vi "onCreateListener.vi"(6 "timeout (ms)":i32=100, 8 "error in (no error)":errorcluster, 10 "Configuration":refnum<class "Connection.TCP-TLS.lvclass">) -> (0 "error out":errorcluster, 3 "Listener":refnum<class "Connection.lvclass">)   [LabVIEW 2020, in "Connection.TCP-TLS.lvclass"]
uses:
  Connection.TCP-TLS.lvclass
  Connection.TCP-TLS.lvclass/Connection.TCP-TLS.ctl
  <vilib>/LabVIEW Open Source Project/MQTT TCP Connection/MQTT_TCP/Connection/TCPConnection.lvclass
  C:/Program Files (x86)/National Instruments/LabVIEW 2020/vi.lib/LabVIEW Open Source Project/MQTT TCP Connection/MQTT_TCP/Connection/TCPConnection.lvclass
  C:/Program Files (x86)/National Instruments/LabVIEW 2020/vi.lib/LabVIEW Open Source Project/MQTT Connection/MQTT_Connection/Connection/Connection.lvclass
  C:/Program Files (x86)/National Instruments/LabVIEW 2020/vi.lib/LabVIEW Open Source Project/Connection/Connection/Connection.lvclass
  C:/Repositories/LVOS/MQTT-Connection-SecuredTCP/source/Connection.SecuredTCP/Connection.TCP-TLS.lvclass
  <vilib>/LabVIEW Open Source Project/Connection/Connection/Connection.lvclass
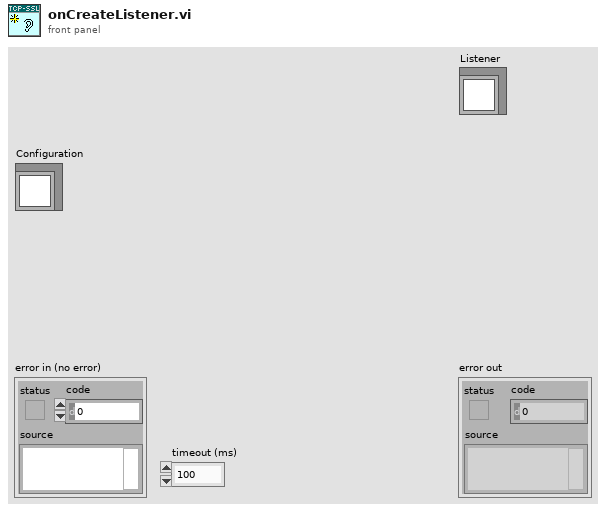
[diagram p1: front panel]
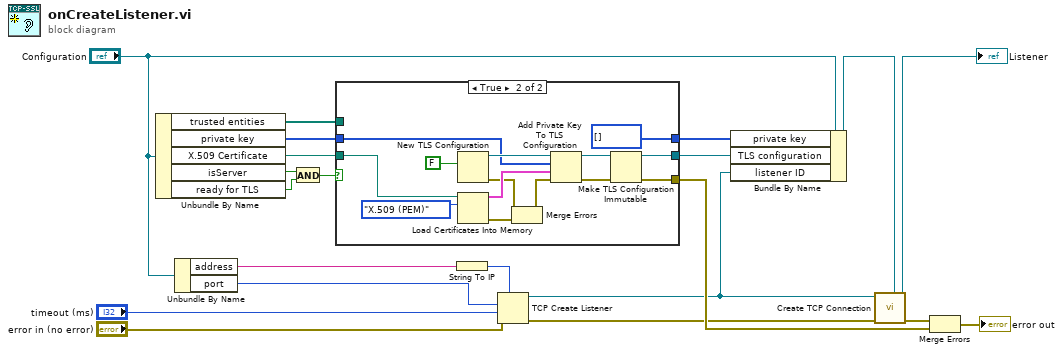
[diagram p0: block diagram]
diagram:
  n1 = Unbundle By Name("Configuration") -> ("trusted entities"=w5:path[], "private key"=w17:u8[], "X.509 Certificate"=w18:path, "isServer"=w4:bool, "ready for TLS"=w2:bool)
  n2 = Unbundle By Name("Configuration") -> ("address"=w19:string, "port"=w21:u16)
  n3 = And(x=w4, y=w2) -> (x .and. y?=w3:bool)
  n4 = case shown="True" w3 {
    tunnel: w18 -> [_ w33]
    tunnel: w17 -> [w22 w32]
    tunnel: [_ w31] -> w16
    tunnel: [_ w27] -> w15
    tunnel: [w22 u8[] [] ("private key")] -> w13
    tunnel: w5 -> [_ _]
    frame False {
    }
    frame True {
      n5 = New TLS Configuration(10:FALSE ("load OS trusted CAs?")) -> (0:w29:errorcluster, 3:w35:refnum<k36>)  [unwired: 1 in]
      n6 = Load Certificates Into Memory(10:enum32{"X.509 (PEM)"}."X.509 (PEM)" ("format"), 11:w33) -> (0:w30:errorcluster, 3:w36:cluster{"certificate":u8[]}[])  [unwired: 1 in]
      n7 = Merge Errors(w29, w30) -> (w28:errorcluster)
      n8 = Add Private Key To TLS Configuration(8:w28, 9:w36, 10:w32, 11:w35) -> (0:w23:errorcluster, 3:w24:refnum<k36>)
      n9 = Make TLS Configuration Immutable(8:w23, 11:w24) -> (0:w27:errorcluster, 3:w31:refnum<k36>)
    }
  }
  n10 = String To IP(1:w19) -> (0:w11:u32)
  n11 = TCP Create Listener(7:w11, 8:"error in (no error)", 9:"timeout (ms)", 10:w21) -> (0:w8:errorcluster, 3:w6:refnum<k5>)  [unwired: 1 in, 1 out]
  n12 = Bundle By Name(cluster="Configuration", "private key"=w13, "TLS configuration"=w16, "listener ID"=w6) -> (w10:refnum<class "Connection.TCP-TLS.lvclass">)
  n13 = call <vilib>:"Create TCP Connection.vi"("TCPConnection in"=w10, "error in (no error)"=w8, "connection ID"=w6) -> ("error out"=w7:errorcluster, "TCPConnection out"=→"Listener":refnum<class "Connection.TCP-TLS.lvclass">)  [unwired: 7 in]
  n14 = Merge Errors(w7, w15) -> (→"error out":errorcluster)
